vi "Receiver_Example - 2 Channel - Experiment_15.vi"() -> ()   [LabVIEW 2022 SP3]
panel:
  in  "stop":bool
  out "BER LP3":dbl
  out "BER HP3":dbl
  out "Inst. BER LP - CH1":dbl format="%#_4g"
  out "OutputHPCH0":i8[](array[numeric])
  out "BER 16QAM":dbl
  out "LP - CH0":dbl format="%#_4g"
  out "Numeric":i32
  out "HP - CH0":dbl format="%#_4g"
  out "x = 0?":bool
  out "iterationsIM":dbl
  in  "State":i32
  in  "Counter":dbl
  in  "Tab Control 3":enum32{"OFDM - 4QAM", "16QAM"}(tab)
  in  "Switch mode":bool
  in  "Tab Control":T1(tab)
  in  "USRP ControledParameters":T2={"Active Antenna"="RX2", "Gain (dB)"=10.0, "Carrier Frequency"=2400000000.0, "IQ Rate"=2000000.0, "Active channels"="0,1"} {"IQ Rate" format="%#_6p"; "Carrier Frequency" format="%#_6p"; "Gain (dB)" format="%#_6f"}
  in  "Device selection":refnum<k15>="RIO0"
  in  "Trigger level":dbl=0.01 format="%f"
  in  "CH0 - LP":T3
  out "CH1 - LP":T3
  out "CH0 - HP":T3
  out "CH1 - HP":T3
  out "SIG valid? - CH1":bool
  out "SIG valid? - CH0":bool
  out "Frequency offset - CH1":dbl
  out "Frequency offset - CH0":dbl
  out "Coerced Parameters":T4={"IQ Rate"=100000.0, "Carrier  Freq."=100000.0, "Gain"=0.0} {"Gain" format="%#_6f"; "Carrier  Freq." format="%#_6p"; "IQ Rate" format="%#_6p"}
  out "Error out":errorcluster
  out "Inst. BER HP - CH0":dbl format="%#_4g"
  out "Acc. BER HP - CH0":dbl format="%#_4g"
  out "Acum. Err HP - CH0":dbl
  out "No. Bits HP - CH0":dbl
  out "Acc. BER LP - CH0":dbl format="%#_4g"
  out "Inst. BER - CH1":dbl format="%#_4g"
  out "Inst. BER LP - CH0":dbl format="%#_4g"
  out "No. Bits - CH1":dbl
  out "No. Bits LP - CH0":dbl
  out "Acum. Err - CH1":dbl
  out "Acum. Err LP - CH0":dbl
  in  "Record BER":bool
  in  "Refresh Button":bool
  out "Acc. BER - CH1":dbl format="%#_4g"
  in  "Boolean 2":bool
  in  "Expected message HP - CH0":string="Critical Dataaaaa\nCritical Dataaaaa\nCritical Dataaaaa\nCritical Dataaaaa\nCritical Dataaaaa"
  out "Expected message HP Detected CH0":string="Non Critical Data\nNon Critical Data\nNon Critical Data\nNon Critical Data\nNon Critical Data"
  in  "Boolean 3":bool
  in  "Boolean":bool
  out "Expected message HP Detected CH1":string="Non Critical Data\nNon Critical Data\nNon Critical Data\nNon Critical Data\nNon Critical Data"
  out "Expected message LP Detected CH0":string="Non Critical Data\nNon Critical Data\nNon Critical Data\nNon Critical Data\nNon Critical Data"
  in  "Expected message - CH1":string="Critical Dataaaaa\nCritical Dataaaaa\nCritical Dataaaaa\nCritical Dataaaaa\nCritical Dataaaaa"
  in  "Expected message LP - CH0":string="Non Critical Data\nNon Critical Data\nNon Critical Data\nNon Critical Data\nNon Critical Data"
  in  "Boolean 5":bool
  in  "Expected message LP - CH1":string="Non Critical Data\nNon Critical Data\nNon Critical Data\nNon Critical Data\nNon Critical Data"
  out "Expected message LP Detected CH1":string="Non Critical Data\nNon Critical Data\nNon Critical Data\nNon Critical Data\nNon Critical Data"
  in  "High-Power Window Size":dbl=15.0 format="%#_6p"
  in  "Low-Power Window Size - CH0":dbl=15.0 format="%#_6p"
  in  "Channel":bool
  in  "Expected message HP - CH0 2":string="Critical Dataaaaa\nCritical Dataaaaa\nCritical Dataaaaa\nCritical Dataaaaa\nCritical Dataaaaa\nNon Critical Data\nNon Critical Data\nNon Critical Data\nNon Critical Data\nNon Critical Data"
  in  "Tab Control 2":enum32{"1 Channel", "2 Channel"}(tab)
  in  "Save data 1 channel":bool
  out "Constellation Map 1 Channel":cdb[](graph)
  out "Low-Power BER - 1 Channel":dbl(graph)
  out "High-Power BER - 1 Channel":dbl(graph)
  out "High-Power Decoded message - 1 Channel":string
  out "Low-Power Decoded message - 1 Channel":string
  out "Low-Power Decoded message - CH0":string
  out "Decoded message - CH1":string
  out "Constellation Map 2 Channel":cluster{"Constellation":cdb[]}[](graph)
  out "Low-Power BER - 2 Channels":T5(graph)
  out "High-Power BER":T6(graph)
  out "High-Power Decoded message - CH0":string
  out "Low-Power Decoded message - CH1":string
  out "CH1 2":bool
  out "CH0 2":bool
  in  "Save data 2 channels":bool
  in  "Color Box 3":u32(colorbox)=11025761
  in  "Color Box 4":u32(colorbox)=7377308
  in  "Save data":bool
  out "Expected message  HP  Detected 2":string="Critical Dataaaaa\nCritical Dataaaaa\nCritical Dataaaaa\nCritical Dataaaaa\nCritical Dataaaaa"
  in  "Boolean 4":bool
  in  "High-Power Window Size 2":dbl=15.0 format="%#_6p"
  out "High-Power Instantaneous BER Graph 2":u8(slide) scale=0.0..100.0
  out "High-Power BER Graph 2":dbl(graph)
  out "No. Bits HP 2":dbl
  out "Acc. BER  HP 2":dbl format="%#_4g"
  out "Acum. Err HP 2":dbl
  out "Inst. BER HP 2":dbl format="%#_4g"
  in  "Expected message 2 HP 2":string="Critical Dataaaaa\nCritical Dataaaaa\nCritical Dataaaaa\nCritical Dataaaaa\nCritical Dataaaaa"
  out "High-Power Decoded Message 2":string
  in  "Record BER 2":bool
  out "Constellation Map 2":cdb[](graph)
  out "Frequency offset 2":dbl
  out "SIG valid? 2":bool
  in  "Refresh Button 2":bool
  out "Error out 2":errorcluster
  in  "error in (no error)":errorcluster
  # "OFDM Superposition Coded Receiver"
  # "Superposition coded\n(criticality-aware)"
  # "Single stream\n(criticality-agnostic)"
  # "1 Channel"
  # "2 Channel"
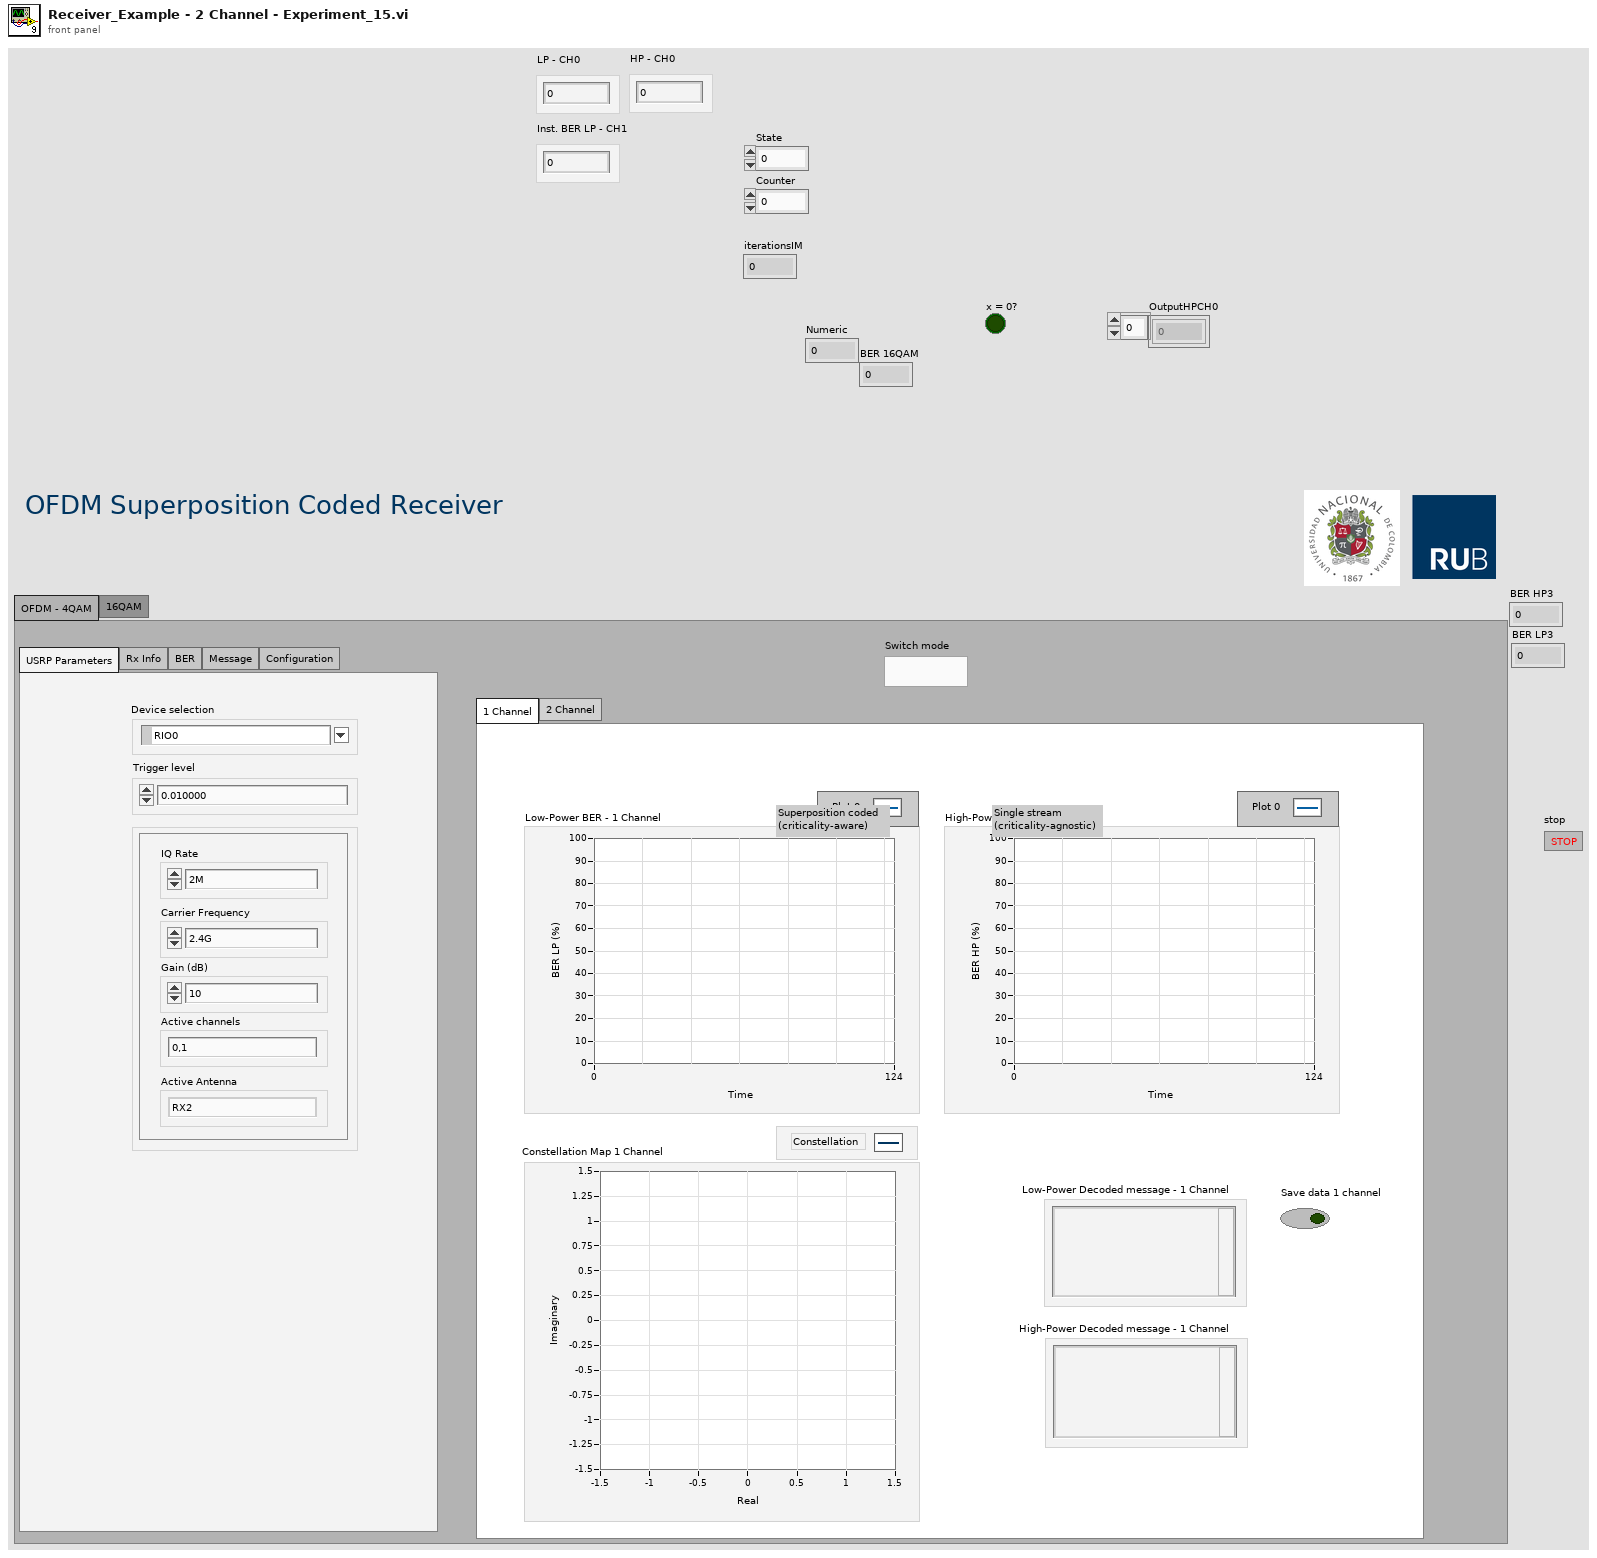
[diagram p1: front panel]
types:
  T1 = enum32{"USRP Parameters", "Rx Info", "BER", "Message", "Configuration"}
  T2 = cluster{"Active Antenna":string, "Gain (dB)":dbl, "Carrier Frequency":dbl, "IQ Rate":dbl, "Active channels":string}
  T3 = cluster{"Modulation type":enum16{"QPSK(4QAM)", "64QAM", "16QAM", "BPSK"}, "BCC rate (k/n)":enum16{"1/2", "2/3", "3/4"}}
  T4 = cluster{"IQ Rate":dbl, "Carrier  Freq.":dbl, "Gain":dbl}
  T5 = cluster{"Graph Instantaneous BER":dbl, "Graph Instantaneous BER":dbl, "Graph Instantaneous BER":dbl}
  T6 = cluster{"Graph Instantaneous BER":dbl, "Graph Instantaneous BER":dbl, "Inst. BER - CH1":dbl}
  T7 = enum16{"open", "replace", "create", "open or create", "replace or create", "replace or create with confirmation"}
  T8 = cluster{"coerced IQ rate":dbl, "coerced carrier frequency":dbl, "coerced gain":dbl}
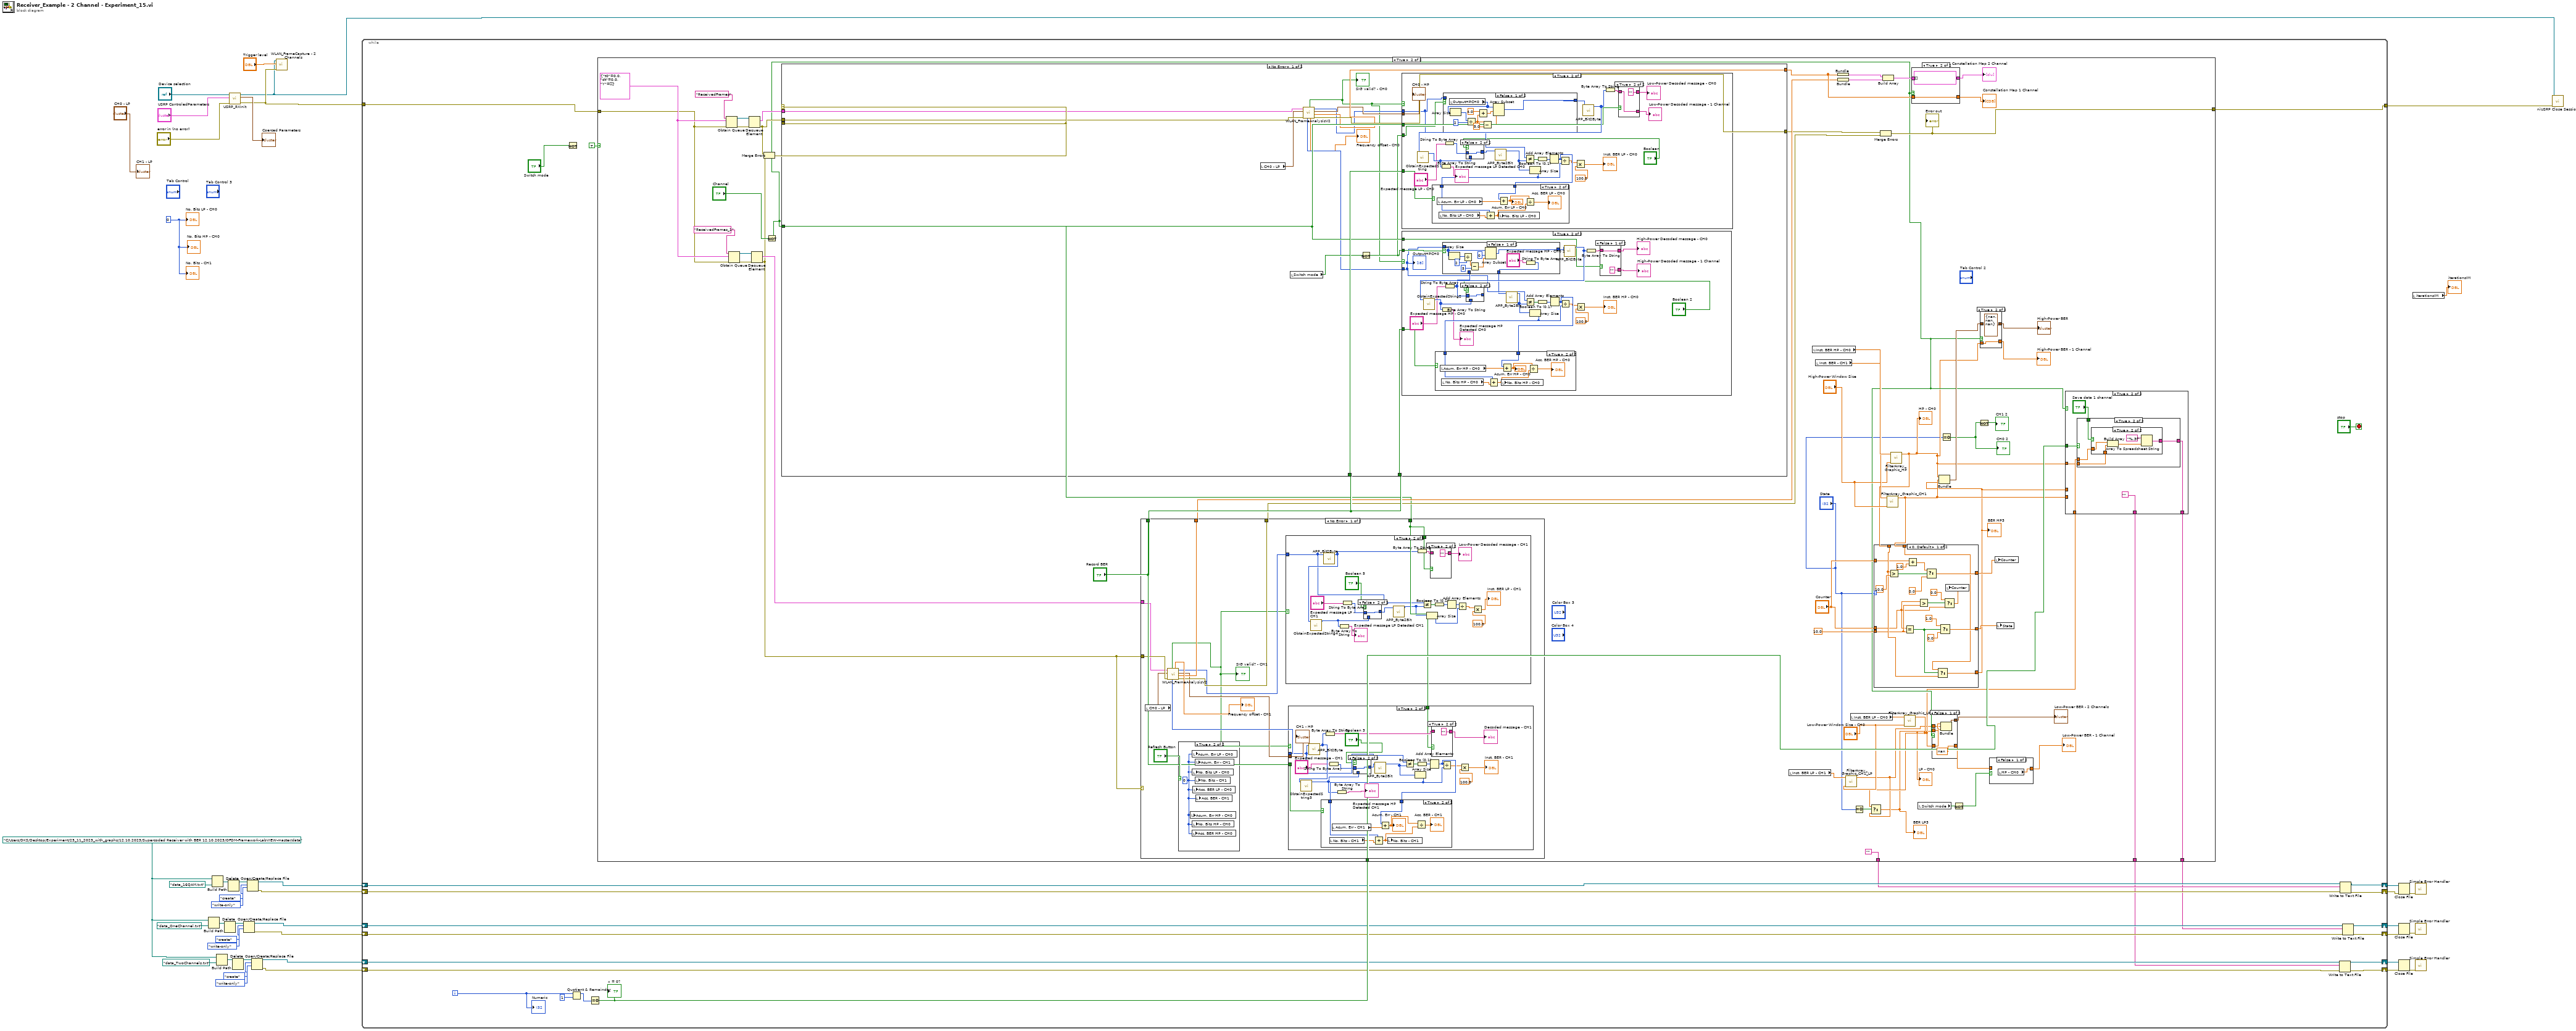
[diagram p0: block diagram]
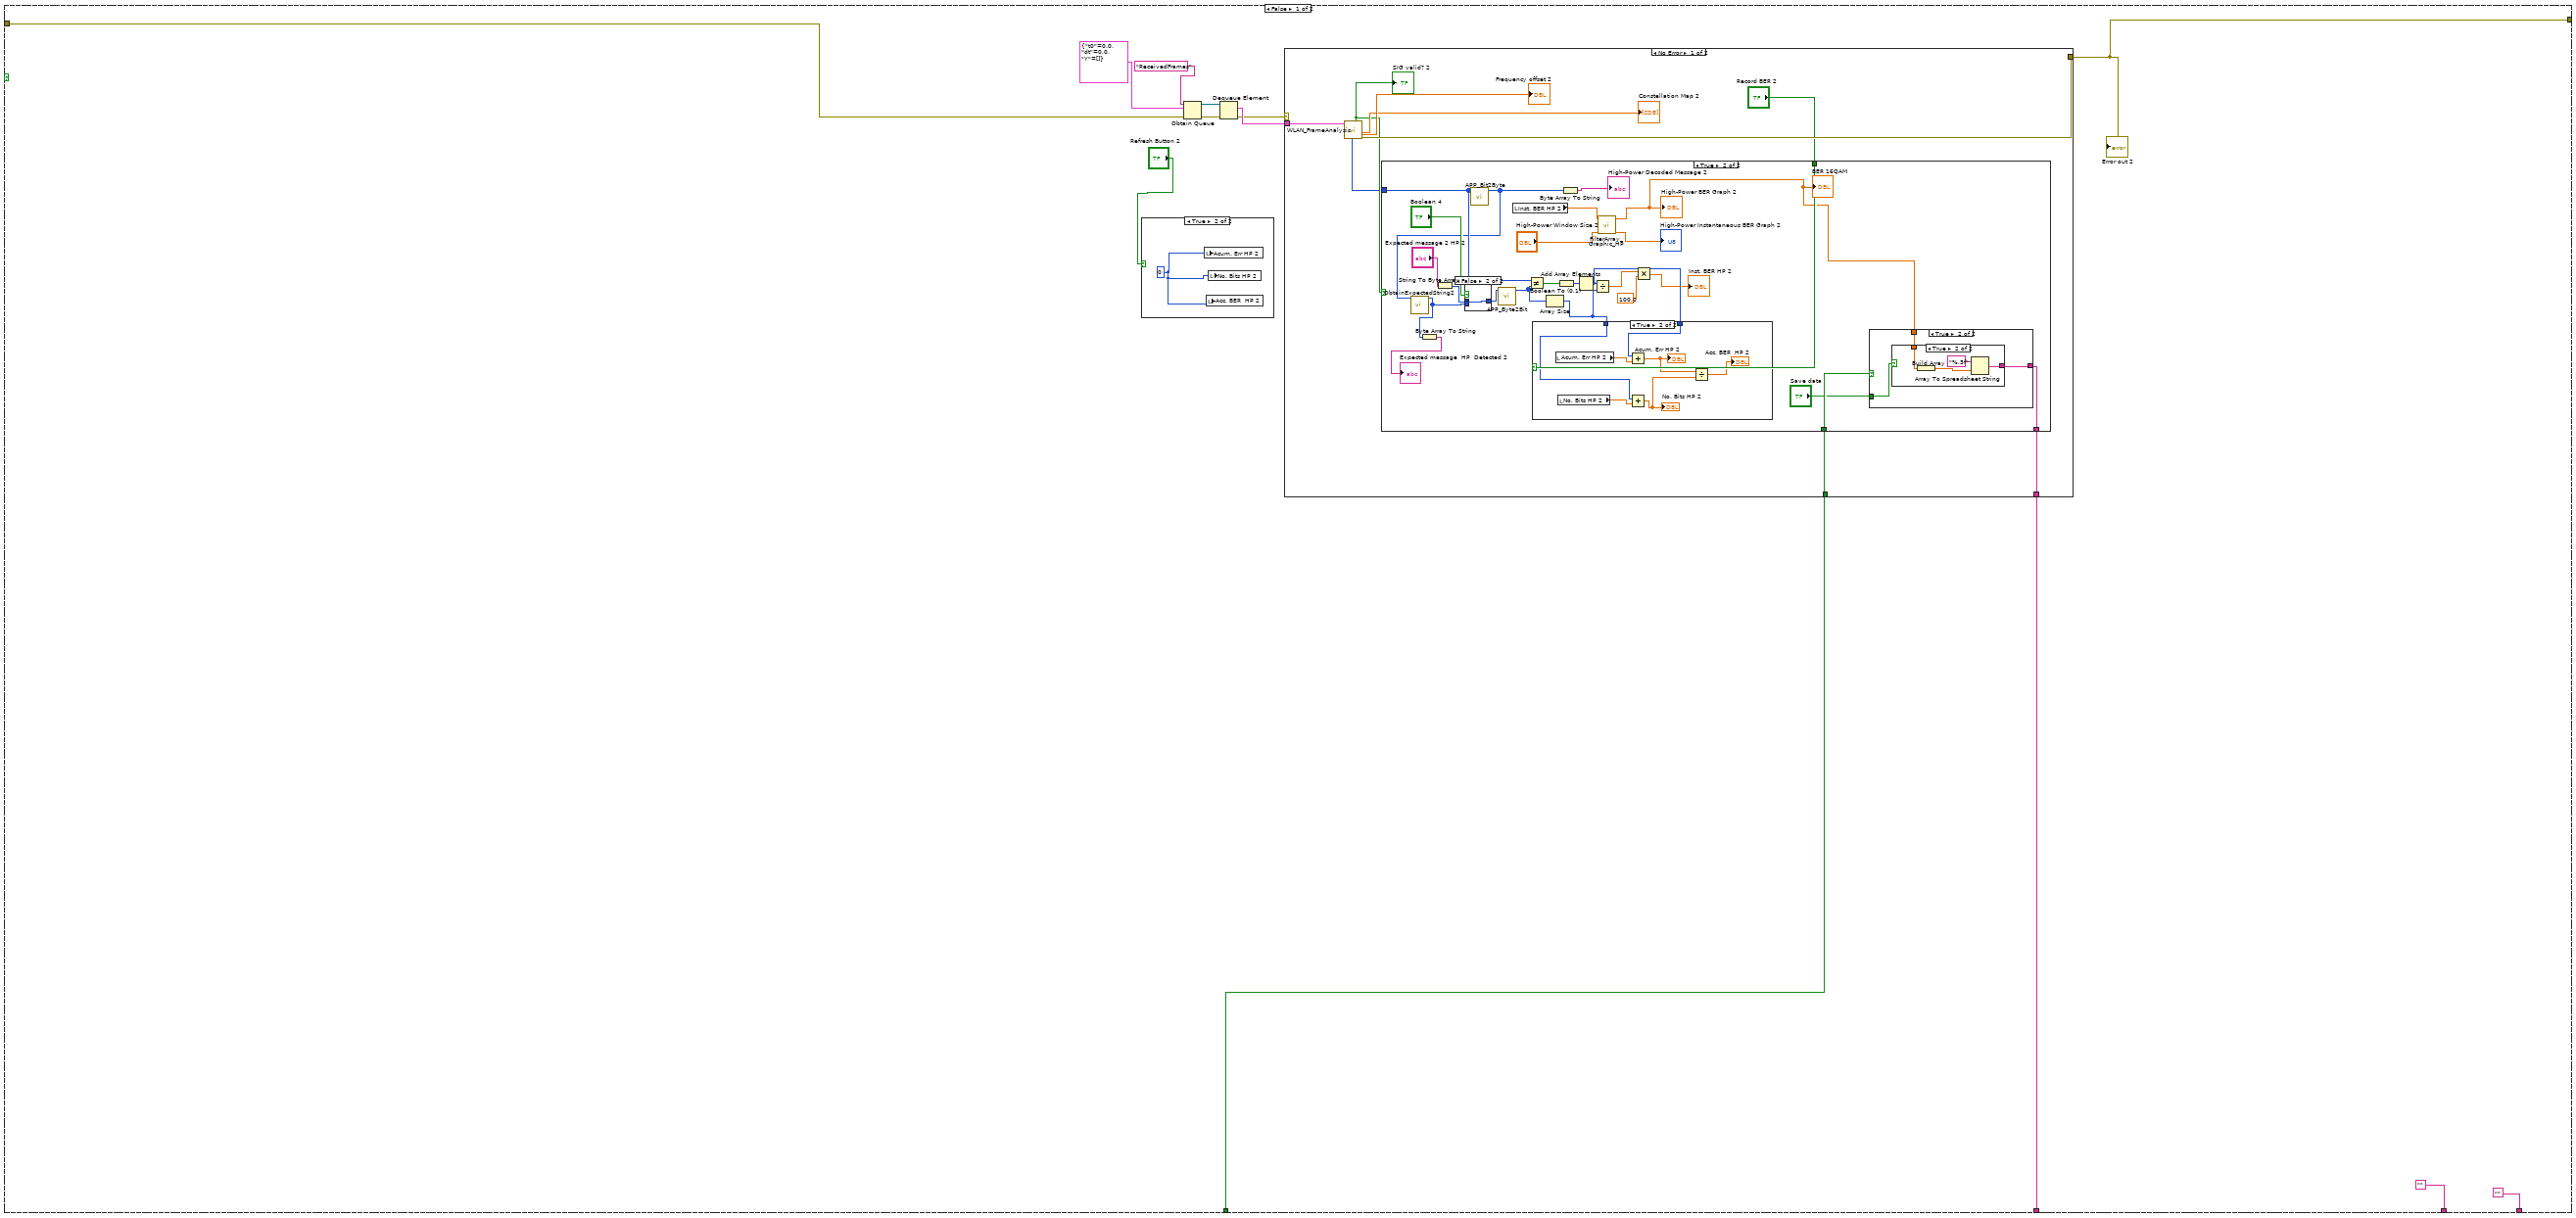
[diagram p2: hidden frame]
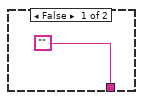
[diagram p4: hidden frame]
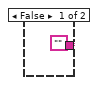
[diagram p5: hidden frame]
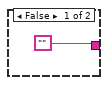
[diagram p6: hidden frame]
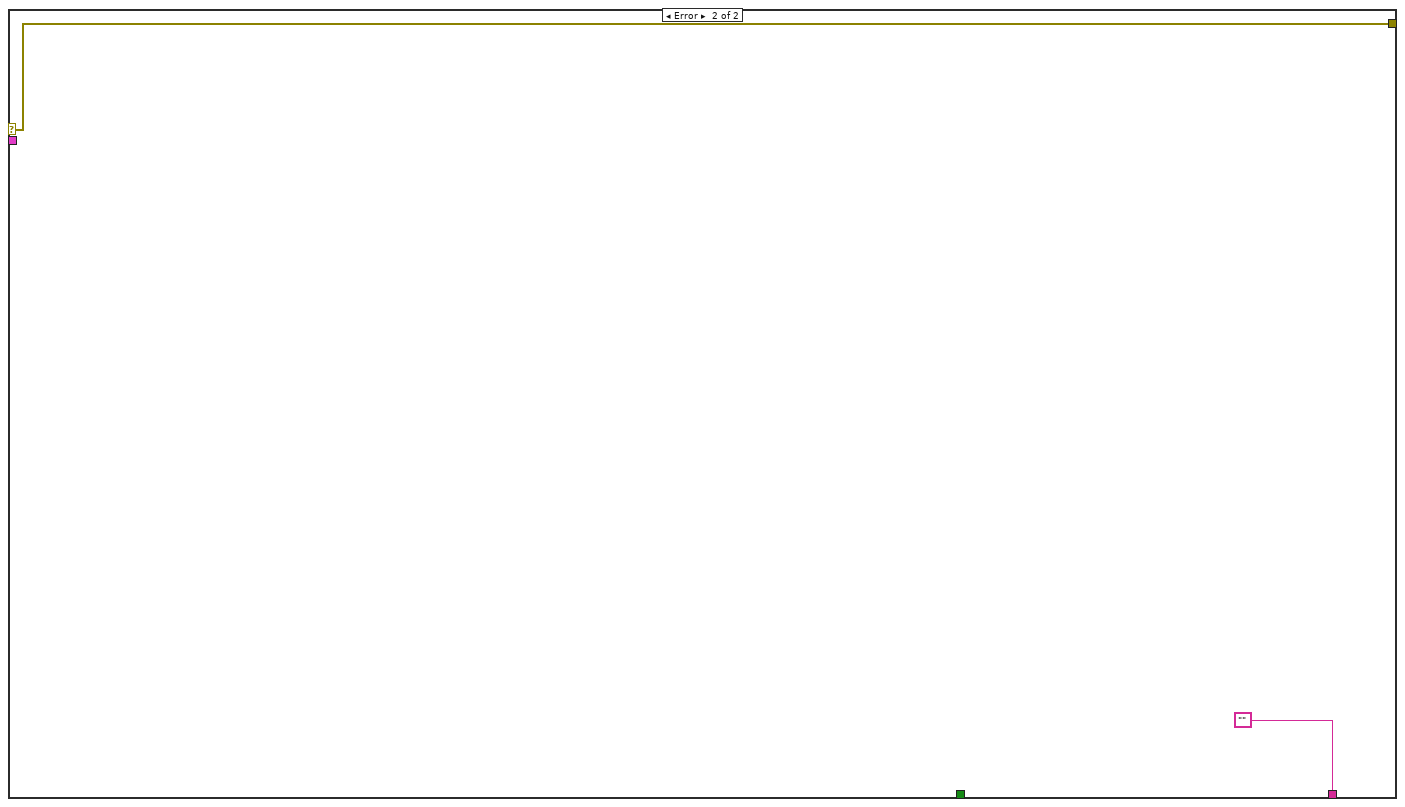
[diagram p9: hidden frame]
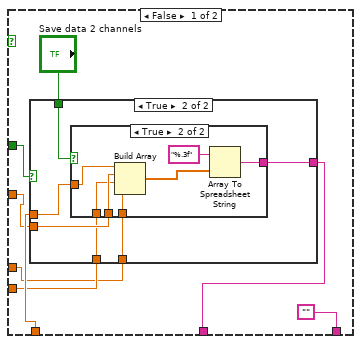
[diagram p11: hidden frame]
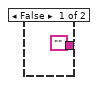
[diagram p12: hidden frame]
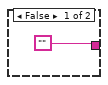
[diagram p13: hidden frame]
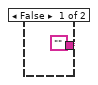
[diagram p14: hidden frame]
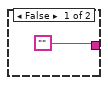
[diagram p15: hidden frame]
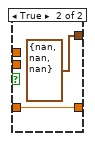
[diagram p16: hidden frame]
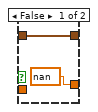
[diagram p17: hidden frame]
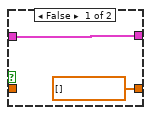
[diagram p18: hidden frame]
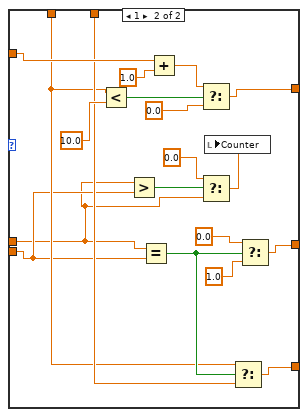
[diagram p19: hidden frame]
diagram:
  w12 = path "C:/Users/DKS/Desktop/Experiment/23_11_2023_with_graphs/12.10.2023/Supercoded Receiver with BER 12.10.2023/OFDM-Framework-LabVIEW-master/data"
  w34 = 0
  n1 = Build Path(base path=w12, name or relative path=path "data_OneChannel.txt" ("default name")) -> (appended path=w22:path)
  n2 = Build Path(base path=w12, name or relative path=path "data_16QAM.txt" ("default name")) -> (appended path=w32:path)
  n3 = Build Path(base path=w12, name or relative path=path "data_TwoChannels.txt" ("default name")) -> (appended path=w17:path)
  n4 = Delete(path (use dialog)=w22) -> (deleted path=w21:path)  [unwired: 4 in, 2 out]
  n5 = Delete(path (use dialog)=w32) -> (deleted path=w31:path)  [unwired: 4 in, 2 out]
  n6 = call "USRP_RXInit.vi"("device names"="Device selection", "USRP ControledParameters"="USRP ControledParameters", "error in (no error)"="error in (no error)") -> ("session handle out"=w37:refnum<k15>, "USRP CoercedParamters"=→"Coerced Parameters":T8, "error out"=w40:errorcluster)  [unwired: 5 in]
  n7 = Delete(path (use dialog)=w17) -> (deleted path=w16:path)  [unwired: 4 in, 2 out]
  n8 = Open/Create/Replace File(file path (use dialog)=w21, operation (0:open)=T7."create", access (0:read/write)=enum16{"read/write", "read-only", "write-only"}."write-only") -> (refnum out=w9:refnum<file>, error out=w8:errorcluster)  [unwired: 1 in, 3 out]
  n9 = Open/Create/Replace File(file path (use dialog)=w31, operation (0:open)=T7."create", access (0:read/write)=enum16{"read/write", "read-only", "write-only"}."write-only") -> (refnum out=w25:refnum<file>, error out=w26:errorcluster)  [unwired: 1 in, 3 out]
  n10 = Open/Create/Replace File(file path (use dialog)=w16, operation (0:open)=T7."create", access (0:read/write)=enum16{"read/write", "read-only", "write-only"}."write-only") -> (refnum out=w7:refnum<file>, error out=w6:errorcluster)  [unwired: 1 in, 3 out]
  n11 = call "WLAN_FrameCapture - 2 Channels.vi"("error in (no error)"=w40, "Trigger level"="Trigger level", "session handle"=w37) -> ()  [unwired: 8 in]
  n12 = while {
    tunnel: w40 -> [w66]
    tunnel: [w65] -> w38
    shift-right: [w61] -> w24
    shift-left: w26 -> [w59]
    shift-right: [w60] -> w23
    shift-left: w25 -> [w58]
    shift-right: [w55] -> w5
    shift-left: w9 -> [w56]
    shift-right: [w53] -> w4
    shift-left: w8 -> [w54]
    shift-right: [w49] -> w3
    shift-left: w7 -> [w52]
    shift-right: [w50] -> w2
    shift-left: w6 -> [w51]
    i -> [w46]
    stop <- "stop" stop-if-true
    n13 = Not(x="Switch mode") -> ()  [unwired: 1 out]
    n14 = Quotient & Remainder(x=w46, y=1) -> (x-y*floor(x/y)=w63:i32)  [unwired: 1 out]
    n15 = Equal To 0?(x=w63) -> (x = 0?=w62:bool)
    "x = 0?" <- w62
    n16 = case shown="True" TRUE {
      tunnel: w66 -> [w72 w159]
      tunnel: [w71 w158] -> w65
      tunnel: w62 -> [w70 w154]
      tunnel: [w69 ""] -> w57
      tunnel: ["" w153] -> w48
      tunnel: ["" w151] -> w47
      frame False {
        n17 = case shown="True" "Refresh Button 2" {
          frame False {
          }
          frame True {
            w80 = 0
            n18 = local write "Acum. Err HP 2"(w80) -> ()
            n19 = local write "Acc. BER  HP 2"(w80) -> ()
            n20 = local write "No. Bits HP 2"(w80) -> ()
          }
        }
        n21 = Obtain Queue(name (unnamed)="ReceivedFrames", element data type=cluster{"t0":dbl, "dt":dbl, "Y":cdb[]} {"t0"=0.0, "dt"=0.0, "Y"=[]} ("data"), error in (no error)=w72) -> (queue out=w73:refnum<queue>, error out=w76:errorcluster)  [unwired: 2 in, 1 out]
        n22 = Dequeue Element(queue=w73, error in (no error)=w76) -> (element=w75:cluster{"t0":dbl, "dt":dbl, "Y":cdb[]}, error out=w74:errorcluster)  [unwired: 1 in, 2 out]
        n23 = case shown="No Error" w74 {
          selector: w74 -> [_ w135]
          tunnel: w75 -> [w88 _]
          tunnel: [w89 w135] -> w71
          tunnel: w70 -> [w82 _]
          tunnel: [w81 ""] -> w69
          frame No Error {
            n24 = call "WLAN_FrameAnalysis.vi"("input cluster"=w88) -> ("error out"=w89:errorcluster, "Constellation"=→"Constellation Map 2":cdb[], "Frequency offset"=→"Frequency offset 2":dbl, "SIG valid?"=w84:bool, "outputbitsHP"=w83:i8[])  [unwired: 4 in, 2 out]
            "SIG valid? 2" <- w84
            n25 = case shown="True" w84 {
              tunnel: "Record BER 2" -> [_ w109]
              tunnel: w83 -> [_ w104]
              tunnel: w82 -> [_ w94]
              tunnel: ["" w92] -> w81
              frame False {
              }
              frame True {
                n26 = String To Byte Array(string="Expected message 2 HP 2") -> (unsigned byte array=w102:u8[])
                n27 = call "APP_Bit2Byte.vi"("input bit stream"=w104) -> ("output byte stream"=w98:u8[])  [unwired: 10 in]
                n28 = call "ObtainExpectedString2.vi"("Array"=w98) -> ("detectedMessage"=w100:i8[])  [unwired: 9 in]
                n29 = Byte Array To String(unsigned byte array=w100) -> (string=→"Expected message  HP  Detected 2":string)
                n30 = case shown="False" "Boolean 4" {
                  tunnel: [w125 w126] -> w103
                  tunnel: w102 -> [_ w126]
                  tunnel: w100 -> [w125 _]
                  frame True {
                  }
                  frame False {
                  }
                }
                n31 = call "APP_Byte2Bit.vi"("input byte stream"=w103) -> ("output bit stream"=w105:i8[])  [unwired: 10 in]
                n32 = local read "Inst. BER HP 2"() -> (w108:dbl)
                n33 = Not Equal?(x=w104, y=w105) -> (x != y?=w113:bool[])
                n34 = Array Size(array=w105) -> (size(s)=w110:i32)
                n35 = Boolean To (0,1)(Boolean=w113) -> (0, 1=w112:i16[])
                n36 = Byte Array To String(unsigned byte array=w98) -> (string=→"High-Power Decoded Message 2":string)
                n37 = Add Array Elements(numeric array=w112) -> (sum=w111:i16)
                n38 = case shown="True" w109 {
                  tunnel: w111 -> [_ w132]
                  tunnel: w110 -> [_ w127]
                  frame False {
                  }
                  frame True {
                    n39 = local read "Acum. Err HP 2"() -> (w133:dbl)
                    n40 = local read "No. Bits HP 2"() -> (w129:dbl)
                    n41 = Add(x=w132, y=w133) -> (x+y=w131:dbl)
                    "Acum. Err HP 2" <- w131
                    n42 = Add(x=w127, y=w129) -> (x+y=w128:dbl)
                    "No. Bits HP 2" <- w128
                    n43 = Divide(x=w131, y=w128) -> (x/y=→"Acc. BER  HP 2":dbl)
                  }
                }
                n44 = Divide(x=w111, y=w110) -> (x/y=w97:dbl)
                n45 = call "FilterArray_Graphic_HP.vi"("Window Size"="High-Power Window Size 2", "Instantaneous BER"=w108) -> ("Slide Bar"=→"High-Power Instantaneous BER Graph 2":dbl, "Graph Instantaneous BER"=w91:dbl)  [unwired: 4 in]
                "High-Power BER Graph 2" <- w91
                "BER 16QAM" <- w91
                n46 = Multiply(x=w97, y=100.0) -> (x*y=→"Inst. BER HP 2":dbl)
                n47 = case shown="True" w94 {
                  tunnel: ["" w119] -> w92
                  tunnel: w91 -> [_ w118]
                  tunnel: "Save data" -> [_ w117]
                  frame False {
                  }
                  frame True {
                    n48 = case shown="True" w117 {
                      tunnel: ["" w122] -> w119
                      tunnel: w118 -> [_ w121]
                      frame False {
                      }
                      frame True {
                        n49 = Build Array(w121) -> (w124:dbl[])
                        n50 = Array To Spreadsheet String(array=w124, 3:"%.3f") -> (spreadsheet string=w122:string)  [unwired: 1 out]
                      }
                    }
                  }
                }
              }
            }
          }
          frame Error {
          }
        }
        "Error out 2" <- w71
      }
      frame True {
        w193 = cluster{"t0":dbl, "dt":dbl, "Y":cdb[]} {"t0"=0.0, "dt"=0.0, "Y"=[]} ("data")
        n51 = Obtain Queue(name (unnamed)="ReceivedFrames", element data type=w193, error in (no error)=w159) -> (queue out=w160:refnum<queue>, error out=w162:errorcluster)  [unwired: 2 in, 1 out]
        n52 = Obtain Queue(name (unnamed)="ReceivedFrames_1", element data type=w193, error in (no error)=w159) -> (queue out=w164:refnum<queue>, error out=w165:errorcluster)  [unwired: 2 in, 1 out]
        n53 = Dequeue Element(queue=w160, error in (no error)=w162) -> (element=w161:cluster{"t0":dbl, "dt":dbl, "Y":cdb[]}, error out=w168:errorcluster)  [unwired: 1 in, 2 out]
        n54 = Dequeue Element(queue=w164, error in (no error)=w165) -> (element=w170:cluster{"t0":dbl, "dt":dbl, "Y":cdb[]}, error out=w136:errorcluster)  [unwired: 1 in, 2 out]
        n55 = Merge Errors(w168, w136) -> (w167:errorcluster)
        n56 = Not(x="Channel") -> (.not. x?=w155:bool)
        n57 = case shown="No Error" w167 {
          tunnel: w161 -> [w369 _]
          tunnel: w167 -> [_ w471]
          tunnel: w168 -> [w368 _]
          tunnel: [w364 dbl[] []] -> w184
          tunnel: [w365 w471] -> w171
          tunnel: "Record BER" -> [w374 _]
          tunnel: "Record BER" -> [w373 _]
          tunnel: w155 -> [w372 _]
          frame No Error {
            n58 = local read "CH0 - LP"() -> (w360:T3)
            n59 = local read "Switch mode"() -> (w371:bool)
            n60 = call "WLAN_FrameAnalysisV2.vi"("error in (no error)"=w368, "Modulation parameter LP"=w360, "input cluster"=w369) -> ("error out"=w365:errorcluster, "Constellation"=w364:cdb[], "Modulation parameter"=w363:T3, "output bits"=w362:i8[], "Frequency offset"=→"Frequency offset - CH0":dbl, "SIG valid?"=w361:bool, "outputbitsHP"=w367:i8[])  [unwired: 2 in]
            "SIG valid? - CH0" <- w361
            n61 = Not(x=w371) -> (.not. x?=w370:bool)
            n62 = case shown="True" w361 {
              tunnel: w362 -> [_ w426]
              tunnel: w363 -> [_ w446]
              tunnel: w373 -> [_ w443]
              tunnel: w372 -> [_ w429]
              tunnel: w370 -> [_ w427]
              frame False {
              }
              frame True {
                n63 = case shown="False" w427 {
                  tunnel: w426 -> [_ w456]
                  tunnel: [w454 w456] -> w428
                  frame False {
                    n64 = local read "OutputHPCH0"() -> (w453:i8[])
                    n65 = Array Size(array=w453) -> (size(s)=w452:i32)
                    n66 = Divide(x=w452, y=2) -> (x/y=w449:dbl)
                    n67 = Add(x=4.0, y=w449) -> (x+y=w451:dbl)
                    n68 = Subtract(x=w449, y=5.0) -> (x-y=w447:dbl)
                    n69 = Array Subset(array=w453, index=w451, length=w447) -> (w454:i8[])
                  }
                  frame True {
                  }
                }
                n70 = String To Byte Array(string="Expected message LP - CH0") -> (unsigned byte array=w436:u8[])
                n71 = call "APP_Bit2Byte.vi"("input bit stream"=w428) -> ("output byte stream"=w435:u8[])  [unwired: 10 in]
                n72 = call "ObtainExpectedString.vi"("Array"=w435) -> ("detectedMessage"=w434:i8[])  [unwired: 9 in]
                n73 = Byte Array To String(unsigned byte array=w434) -> (string=→"Expected message LP Detected CH0":string)
                n74 = case shown="False" "Boolean" {
                  tunnel: [w461 w462] -> w438
                  tunnel: w436 -> [_ w462]
                  tunnel: w434 -> [w461 _]
                  frame True {
                  }
                  frame False {
                  }
                }
                n75 = call "APP_Byte2Bit.vi"("input byte stream"=w438) -> ("output bit stream"=w437:i8[])  [unwired: 10 in]
                n76 = Not Equal?(x=w426, y=w437) -> (x != y?=w444:bool[])
                n77 = Array Size(array=w437) -> (size(s)=w442:i32)
                n78 = Boolean To (0,1)(Boolean=w444) -> (0, 1=w445:i16[])
                n79 = Add Array Elements(numeric array=w445) -> (sum=w441:i16)
                n80 = case shown="True" w443 {
                  tunnel: w442 -> [_ w468]
                  tunnel: w441 -> [_ w466]
                  frame False {
                  }
                  frame True {
                    n81 = local read "Acum. Err LP - CH0"() -> (w467:dbl)
                    n82 = local read "No. Bits LP - CH0"() -> (w469:dbl)
                    n83 = Add(x=w468, y=w469) -> (x+y=w465:dbl)
                    n84 = Add(x=w466, y=w467) -> (x+y=w464:dbl)
                    "Acum. Err LP - CH0" <- w464
                    n85 = local write "No. Bits LP - CH0"(w465) -> ()
                    n86 = Divide(x=w464, y=w465) -> (x/y=→"Acc. BER LP - CH0":dbl)
                  }
                }
                n87 = Divide(x=w441, y=w442) -> (x/y=w440:dbl)
                n88 = Multiply(x=w440, y=100.0) -> (x*y=→"Inst. BER LP - CH0":dbl)
                n89 = Byte Array To String(unsigned byte array=w435) -> (string=w432:string)
                n90 = case shown="True" w429 {
                  tunnel: w432 -> [w458 w460]
                  tunnel: ["" ("string") w460] -> w431
                  tunnel: [w458 "" ("string")] -> w430
                  frame False {
                  }
                  frame True {
                  }
                }
                "Low-Power Decoded message - CH0" <- w430
                "Low-Power Decoded message - 1 Channel" <- w431
                "CH0 - HP" <- w446
              }
            }
            n91 = case shown="True" w361 {
              tunnel: w367 -> [_ w379]
              tunnel: w374 -> [_ w395]
              tunnel: w372 -> [_ w384]
              tunnel: w370 -> [_ w382]
              frame False {
              }
              frame True {
                n92 = String To Byte Array(string="Expected message HP - CH0") -> (unsigned byte array=w381:u8[])
                n93 = case shown="False" w382 {
                  tunnel: w379 -> [w405 w409]
                  tunnel: [w406 w409] -> w383
                  tunnel: [w398 w408] -> w378
                  tunnel: w381 -> [_ w408]
                  frame False {
                    n94 = Array Size(array=w405) -> (size(s)=w402:i32)
                    n95 = Divide(x=w402, y=2) -> (x/y=w401:dbl)
                    n96 = Subtract(x=w401, y=5) -> (x-y=w403:dbl)
                    n97 = Array Subset(array=w405, index=0, length=w403) -> (w406:i8[])
                    n98 = String To Byte Array(string="Expected message HP - CH0 2") -> (unsigned byte array=w398:u8[])
                  }
                  frame True {
                  }
                }
                n99 = call "APP_Byte2Bit.vi"("input byte stream"=w378) -> ("output bit stream"=w380:i8[])  [unwired: 10 in]
                n100 = Not Equal?(x=w379, y=w380) -> (x != y?=w396:bool[])
                n101 = Array Size(array=w380) -> (size(s)=w394:i32)
                n102 = Boolean To (0,1)(Boolean=w396) -> (0, 1=w397:i16[])
                n103 = Add Array Elements(numeric array=w397) -> (sum=w393:i16)
                n104 = case shown="True" w395 {
                  tunnel: w394 -> [_ w421]
                  tunnel: w393 -> [_ w419]
                  frame False {
                  }
                  frame True {
                    n105 = local read "Acum. Err HP - CH0"() -> (w420:dbl)
                    n106 = local read "No. Bits HP - CH0"() -> (w422:dbl)
                    n107 = Add(x=w421, y=w422) -> (x+y=w418:dbl)
                    n108 = local write "No. Bits HP - CH0"(w418) -> ()
                    n109 = Add(x=w419, y=w420) -> (x+y=w417:dbl)
                    "Acum. Err HP - CH0" <- w417
                    n110 = Divide(x=w417, y=w418) -> (x/y=→"Acc. BER HP - CH0":dbl)
                  }
                }
                n111 = Divide(x=w393, y=w394) -> (x/y=w392:dbl)
                n112 = call "APP_Bit2Byte.vi"("input bit stream"=w383) -> ("output byte stream"=w390:u8[])  [unwired: 10 in]
                n113 = call "ObtainExpectedString2.vi"("Array"=w390) -> ("detectedMessage"=w389:i8[])  [unwired: 9 in]
                n114 = Byte Array To String(unsigned byte array=w389) -> (string=→"Expected message HP Detected CH0":string)
                n115 = case shown="False" "Boolean 2" {
                  tunnel: [w414 w415] -> _
                  tunnel: w381 -> [_ w415]
                  tunnel: w389 -> [w414 _]
                  frame True {
                  }
                  frame False {
                  }
                }
                n116 = Multiply(x=w392, y=100.0) -> (x*y=→"Inst. BER HP - CH0":dbl)
                n117 = Byte Array To String(unsigned byte array=w390) -> (string=w385:string)
                n118 = case shown="False" w384 {
                  tunnel: w385 -> [w411 w413]
                  tunnel: ["" ("string") w413] -> w386
                  tunnel: [w411 "" ("string")] -> w387
                  frame False {
                  }
                  frame True {
                  }
                }
                "High-Power Decoded message - CH0" <- w387
                "High-Power Decoded message - 1 Channel" <- w386
                "OutputHPCH0" <- w379
              }
            }
          }
          frame Error {
          }
        }
        n119 = case shown="No Error" w136 {
          tunnel: w170 -> [w297 _]
          tunnel: "Record BER" -> [w300 _]
          tunnel: [w294 w358] -> w172
          tunnel: [w293 dbl[] []] -> w173
          tunnel: w155 -> [w299 _]
          tunnel: w136 -> [w298 w358]
          frame No Error {
            n120 = local read "CH0 - LP"() -> (w289:T3)
            n121 = call "WLAN_FrameAnalysisV2.vi"("error in (no error)"=w298, "Modulation parameter LP"=w289, "input cluster"=w297) -> ("error out"=w294:errorcluster, "Constellation"=w293:cdb[], "Modulation parameter"=w292:T3, "output bits"=w291:i8[], "Frequency offset"=→"Frequency offset - CH1":dbl, "SIG valid?"=w290:bool, "outputbitsHP"=w296:i8[])  [unwired: 2 in]
            "SIG valid? - CH1" <- w290
            n122 = case shown="True" "Refresh Button" {
              frame False {
              }
              frame True {
                w325 = 0
                n123 = local write "Acum. Err HP - CH0"(w325) -> ()
                n124 = local write "Acc. BER HP - CH0"(w325) -> ()
                n125 = local write "Acum. Err LP - CH0"(w325) -> ()
                n126 = local write "No. Bits LP - CH0"(w325) -> ()
                n127 = local write "No. Bits HP - CH0"(w325) -> ()
                n128 = local write "Acc. BER LP - CH0"(w325) -> ()
                n129 = local write "Acum. Err - CH1"(w325) -> ()
                n130 = local write "No. Bits - CH1"(w325) -> ()
                n131 = local write "Acc. BER - CH1"(w325) -> ()
              }
            }
            n132 = case shown="True" w290 {
              tunnel: w291 -> [_ w303]
              tunnel: w299 -> [_ w318]
              frame False {
              }
              frame True {
                n133 = call "APP_Bit2Byte.vi"("input bit stream"=w303) -> ("output byte stream"=w313:u8[])  [unwired: 10 in]
                n134 = call "ObtainExpectedString4.vi"("Array"=w313) -> ("detectedMessage"=w314:i8[])  [unwired: 9 in]
                n135 = Byte Array To String(unsigned byte array=w314) -> (string=→"Expected message LP Detected CH1":string)
                n136 = String To Byte Array(string="Expected message LP - CH1") -> (unsigned byte array=w317:u8[])
                n137 = case shown="False" "Boolean 5" {
                  tunnel: [w321 w322] -> w312
                  tunnel: w317 -> [_ w322]
                  tunnel: w314 -> [w321 _]
                  frame True {
                  }
                  frame False {
                  }
                }
                n138 = call "APP_Byte2Bit.vi"("input byte stream"=w312) -> ("output bit stream"=w304:i8[])  [unwired: 10 in]
                n139 = Byte Array To String(unsigned byte array=w313) -> (string=w320:string)
                n140 = Not Equal?(x=w303, y=w304) -> (x != y?=w310:bool[])
                n141 = Array Size(array=w304) -> (size(s)=w309:i32)
                n142 = case shown="True" w318 {
                  tunnel: w320 -> [w323 _]
                  tunnel: [w323 "" ("string")] -> w319
                  frame False {
                  }
                  frame True {
                  }
                }
                "Low-Power Decoded message - CH1" <- w319
                n143 = Boolean To (0,1)(Boolean=w310) -> (0, 1=w311:i16[])
                n144 = Add Array Elements(numeric array=w311) -> (sum=w308:i16)
                n145 = Divide(x=w308, y=w309) -> (x/y=w307:dbl)
                n146 = Multiply(x=w307, y=100.0) -> (x*y=→"Inst. BER LP - CH1":dbl)
              }
            }
            n147 = case shown="True" w290 {
              tunnel: w296 -> [_ w334]
              tunnel: w292 -> [_ w346]
              tunnel: w300 -> [_ w332]
              tunnel: w299 -> [_ w329]
              frame False {
              }
              frame True {
                n148 = call "APP_Bit2Byte.vi"("input bit stream"=w334) -> ("output byte stream"=w336:u8[])  [unwired: 10 in]
                n149 = call "ObtainExpectedString3.vi"("Array"=w336) -> ("detectedMessage"=w335:i8[])  [unwired: 9 in]
                n150 = Byte Array To String(unsigned byte array=w336) -> (string=w330:string)
                n151 = String To Byte Array(string="Expected message - CH1") -> (unsigned byte array=w337:u8[])
                n152 = Byte Array To String(unsigned byte array=w335) -> (string=→"Expected message HP Detected CH1":string)
                n153 = case shown="False" "Boolean 3" {
                  tunnel: [w349 w350] -> w339
                  tunnel: w337 -> [_ w350]
                  tunnel: w335 -> [w349 _]
                  frame True {
                  }
                  frame False {
                  }
                }
                n154 = call "APP_Byte2Bit.vi"("input byte stream"=w339) -> ("output bit stream"=w338:i8[])  [unwired: 10 in]
                n155 = Not Equal?(x=w334, y=w338) -> (x != y?=w344:bool[])
                n156 = Array Size(array=w338) -> (size(s)=w343:i32)
                n157 = Boolean To (0,1)(Boolean=w344) -> (0, 1=w345:i16[])
                n158 = Add Array Elements(numeric array=w345) -> (sum=w342:i16)
                n159 = case shown="True" w332 {
                  tunnel: w343 -> [_ w356]
                  tunnel: w342 -> [_ w354]
                  frame False {
                  }
                  frame True {
                    n160 = local read "No. Bits - CH1"() -> (w357:dbl)
                    n161 = local read "Acum. Err - CH1"() -> (w355:dbl)
                    n162 = Add(x=w356, y=w357) -> (x+y=w353:dbl)
                    n163 = Add(x=w354, y=w355) -> (x+y=w352:dbl)
                    "Acum. Err - CH1" <- w352
                    n164 = local write "No. Bits - CH1"(w353) -> ()
                    n165 = Divide(x=w352, y=w353) -> (x/y=→"Acc. BER - CH1":dbl)
                  }
                }
                n166 = case shown="True" w329 {
                  tunnel: w330 -> [w347 _]
                  tunnel: [w347 "" ("string")] -> w331
                  frame False {
                  }
                  frame True {
                  }
                }
                "Decoded message - CH1" <- w331
                n167 = Divide(x=w342, y=w343) -> (x/y=w340:dbl)
                n168 = Multiply(x=w340, y=100.0) -> (x*y=→"Inst. BER - CH1":dbl)
                "CH1 - HP" <- w346
              }
            }
          }
          frame Error {
          }
        }
        n169 = local read "Inst. BER LP - CH1"() -> (w143:dbl)
        n170 = local read "Inst. BER HP - CH0"() -> (w189:dbl)
        n171 = local read "Inst. BER - CH1"() -> (w180:dbl)
        n172 = Bundle("Constellation"=w184) -> (w183:cluster{"Constellation":cdb[]})  [unwired: 1 in]
        n173 = Bundle("Constellation"=w173) -> (w169:cluster{"Constellation":cdb[]})  [unwired: 1 in]
        n174 = call "FilterArray_Graphic_CH1_LP.vi"("Window Size"="Low-Power Window Size - CH0", "Instantaneous BER"=w143) -> ("Graph Instantaneous BER"=w138:dbl)  [unwired: 4 in, 1 out]
        n175 = local read "Inst. BER LP - CH0"() -> (w156:dbl)
        n176 = Equal To 0?(x="State") -> (x = 0?=w141:bool)
        n177 = Merge Errors(w171, w172) -> (w158:errorcluster)
        "Error out" <- w158
        n178 = Build Array(w183, w169) -> (w186:cluster{"Constellation":cdb[]}[])
        n179 = call "FilterArray_Graphic_CH1.vi"("Window Size"="High-Power Window Size", "Instantaneous BER"=w180) -> ("Graph Instantaneous BER"=w152:dbl)  [unwired: 4 in, 1 out]
        n180 = call "FilterArray_Graphic_HP.vi"("Window Size"="High-Power Window Size", "Instantaneous BER"=w189) -> ("Graph Instantaneous BER"=w149:dbl)  [unwired: 4 in, 1 out]
        "HP - CH0" <- w149
        n181 = case shown="0, Default" "State" {
          tunnel: "Counter" -> [w257 w277]
          tunnel: [w264 w280] -> w176
          tunnel: "Counter" -> [w252 w270]
          tunnel: [w261 w279] -> w177
          tunnel: [w259 w278] -> w150
          tunnel: w149 -> [w258 w275]
          tunnel: w152 -> [w256 w276]
          tunnel: 10.0 ("y") -> [w255 w271]
          frame 0, Default {
            n182 = Greater?(x=w258, y=10.0) -> (0:w265:bool)
            n183 = Equal?(x=w252, y=w255) -> (x = y?=w260:bool)
            n184 = Add(x=w257, y=1.0) -> (x+y=w267:dbl)
            n185 = Greater?(x=w252, y=w255) -> (0:w254:bool)
            n186 = Select(t=w267, s=w265, f=0.0) -> (s? t:f=w264:dbl)
            n187 = Select(t=w256, s=w260, f=w258) -> (s? t:f=w259:dbl)
            n188 = Select(t=1.0, s=w260, f=0.0) -> (s? t:f=w261:dbl)
            n189 = Select(t=0.0, s=w254, f=w252) -> (s? t:f=w251:dbl)
            n190 = local write "Counter"(w251) -> ()
          }
          frame 1 {
            n191 = Less?(x=w275, y=10.0) -> (x < y?=w281:bool)
            n192 = Greater?(x=w270, y=w271) -> (0:w273:bool)
            n193 = Equal?(x=w270, y=w271) -> (x = y?=w283:bool)
            n194 = Add(x=w277, y=1.0) -> (x+y=w287:dbl)
            n195 = Select(t=w287, s=w281, f=0.0) -> (s? t:f=w280:dbl)
            n196 = Select(t=0.0, s=w273, f=w270) -> (s? t:f=w274:dbl)
            n197 = local write "Counter"(w274) -> ()
            n198 = Select(t=w275, s=w283, f=w276) -> (s? t:f=w278:dbl)
            n199 = Select(t=0.0, s=w283, f=1.0) -> (s? t:f=w279:dbl)
          }
        }
        "BER HP3" <- w150
        n200 = call "FilterArray_Graphic_LP.vi"("Window Size"="Low-Power Window Size - CH0", "Instantaneous BER"=w156) -> ("Graph Instantaneous BER"=w139:dbl)  [unwired: 4 in, 1 out]
        "LP - CH0" <- w139
        n201 = Select(t=w139, s=w141, f=w138) -> (s? t:f=w137:dbl)
        "BER LP3" <- w137
        n202 = case shown="True" w155 {
          tunnel: [cdb[] [] ("Constellation") w250] -> w185
          tunnel: w184 -> [_ w250]
          tunnel: w186 -> [w248 _]
          tunnel: [w248 cluster{"Constellation":cdb[]}[] []] -> w187
          frame False {
          }
          frame True {
          }
        }
        "Constellation Map 2 Channel" <- w187
        "Constellation Map 1 Channel" <- w185
        n203 = local read "Switch mode"() -> (w148:bool)
        n204 = case shown="False" w155 {
          tunnel: w139 -> [w238 w242]
          tunnel: [nan ("Graph Instantaneous BER") w242] -> w145
          tunnel: [w239 T5 {"Graph Instantaneous BER"=nan, "Graph Instantaneous BER"=nan, "Graph Instantaneous BER"=nan}] -> w146
          tunnel: w138 -> [w237 _]
          tunnel: w137 -> [w236 _]
          frame False {
            n205 = Bundle("Graph Instantaneous BER"=w238, "Graph Instantaneous BER"=w237, "Graph Instantaneous BER"=w236) -> (w239:T5)  [unwired: 1 in]
          }
          frame True {
          }
        }
        "Low-Power BER - 2 Channels" <- w146
        n206 = Bundle("Graph Instantaneous BER"=w149, "Graph Instantaneous BER"=w152, "Graph Instantaneous BER"=w150) -> (w191:T5)  [unwired: 1 in]
        n207 = Equal To 0?(x="State") -> (x = 0?=w182:bool)
        "CH0 2" <- w182
        n208 = Not(x=w148) -> (.not. x?=w147:bool)
        n209 = Not(x=w182) -> (.not. x?=→"CH1 2":bool)
        n210 = case shown="True" w155 {
          tunnel: w149 -> [_ w246]
          tunnel: [nan w246] -> w190
          tunnel: w191 -> [w244 _]
          tunnel: [w244 T5 {"Graph Instantaneous BER"=nan, "Graph Instantaneous BER"=nan, "Graph Instantaneous BER"=nan}] -> w192
          frame False {
          }
          frame True {
          }
        }
        "High-Power BER" <- w192
        "High-Power BER - 1 Channel" <- w190
        n211 = case shown="False" w147 {
          tunnel: w145 -> [_ w195]
          tunnel: [w194 w195] -> w144
          frame False {
            n212 = local read "HP - CH0"() -> (w194:dbl)
          }
          frame True {
          }
        }
        "Low-Power BER - 1 Channel" <- w144
        n213 = local write "Counter"(w176) -> ()
        n214 = local write "State"(w177) -> ()
        n215 = case shown="True" w155 {
          tunnel: w139 -> [w200 w224]
          tunnel: w149 -> [w199 w223]
          tunnel: w154 -> [w202 w222]
          tunnel: ["" w220] -> w153
          tunnel: w152 -> [w198 _]
          tunnel: w150 -> [w197 _]
          tunnel: [w196 ""] -> w151
          frame False {
            n216 = case shown="True" w202 {
              tunnel: ["" w210] -> w196
              tunnel: w200 -> [_ w208]
              tunnel: w199 -> [_ w209]
              tunnel: "Save data 2 channels" -> [_ w207]
              tunnel: w198 -> [_ w206]
              tunnel: w197 -> [_ w205]
              frame False {
              }
              frame True {
                n217 = case shown="True" w207 {
                  tunnel: ["" w216] -> w210
                  tunnel: w208 -> [_ w215]
                  tunnel: w209 -> [_ w214]
                  tunnel: w206 -> [_ w213]
                  tunnel: w205 -> [_ w212]
                  frame False {
                  }
                  frame True {
                    n218 = Build Array(w215, w214, w213, w212) -> (w218:dbl[])
                    n219 = Array To Spreadsheet String(array=w218, 3:"%.3f") -> (spreadsheet string=w216:string)  [unwired: 1 out]
                  }
                }
              }
            }
          }
          frame True {
            n220 = case shown="True" w222 {
              tunnel: ["" w229] -> w220
              tunnel: w224 -> [_ w227]
              tunnel: w223 -> [_ w228]
              tunnel: "Save data 1 channel" -> [_ w226]
              frame False {
              }
              frame True {
                n221 = case shown="True" w226 {
                  tunnel: ["" w233] -> w229
                  tunnel: w227 -> [_ w232]
                  tunnel: w228 -> [_ w231]
                  frame False {
                  }
                  frame True {
                    n222 = Build Array(w232, w231) -> (w235:dbl[])
                    n223 = Array To Spreadsheet String(array=w235, 3:"%.3f") -> (spreadsheet string=w233:string)  [unwired: 1 out]
                  }
                }
              }
            }
          }
        }
      }
    }
    n224 = Write to Text File(file (use dialog)=w52, text=w47, error in=w51) -> (refnum out=w49:refnum<file>, error out=w50:errorcluster)  [unwired: 1 in, 1 out]
    n225 = Write to Text File(file (use dialog)=w58, text=w57, error in=w59) -> (refnum out=w60:refnum<file>, error out=w61:errorcluster)  [unwired: 1 in, 1 out]
    n226 = Write to Text File(file (use dialog)=w56, text=w48, error in=w54) -> (refnum out=w55:refnum<file>, error out=w53:errorcluster)  [unwired: 1 in, 1 out]
    "Numeric" <- w46
  }
  n227 = Close File(refnum=w23, error in=w24) -> (error out=w27:errorcluster)  [unwired: 1 out]
  n228 = Close File(refnum=w5, error in=w4) -> (error out=w11:errorcluster)  [unwired: 1 out]
  n229 = Close File(refnum=w3, error in=w2) -> (error out=w10:errorcluster)  [unwired: 1 out]
  n230 = local read "iterationsIM"() -> (→"iterationsIM":dbl)
  n231 = call <vilib>:"Simple Error Handler.vi"("error in (no error)"=w27) -> ()  [unwired: 1 in, 8 out]
  n232 = call <vilib>:"Simple Error Handler.vi"("error in (no error)"=w11) -> ()  [unwired: 1 in, 8 out]
  n233 = call <vilib>:"Simple Error Handler.vi"("error in (no error)"=w10) -> ()  [unwired: 1 in, 8 out]
  n234 = call <instrlib>:"niUSRP Close Session.vi"("session handle"=w37, "error in (no error)"=w38) -> ()  [unwired: 13 in, 1 out]
  "No. Bits LP - CH0" <- w34
  "No. Bits - CH1" <- w34
  "No. Bits HP - CH0" <- w34
  "CH1 - LP" <- "CH0 - LP"
